vi "Update Stats.vi"(6 "ACK Errors":u32, 8 "error in (no error)":errorcluster, 9 "Number Read":i32, 10 "Number Filtered":u32, 11 "CAN_RW_CORE in":refnum<class "CAN_RW_CORE.lvclass">) -> (0 "error out":errorcluster, 3 "CAN_RW_CORE out":refnum<class "CAN_RW_CORE.lvclass">)   [LabVIEW 2021, in "CAN_RW_CORE.lvclass"]
uses:
  CAN_RW_CORE.lvclass
  CAN_RW_CORE.lvclass/CAN_RW_CORE.ctl
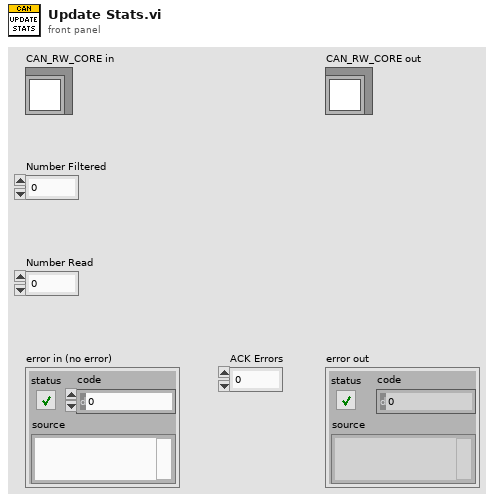
[diagram p1: front panel]
types:
  T1 = typedef "CAN_RW_CORE.lvclass/Statistics.ctl" = cluster{"Total Frames RW":u32, "Frames Filtered ":u32, "ACK Errors":u32}
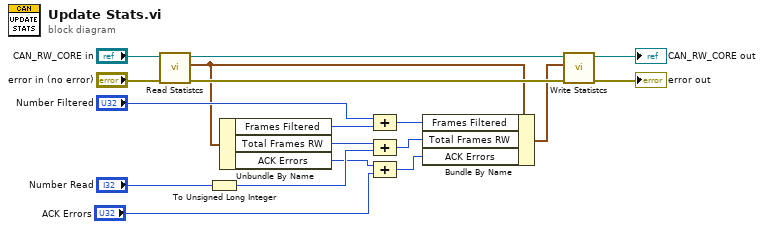
[diagram p0: block diagram]
diagram:
  n1 = call "Read Statistcs.vi"("error in (no error)"="error in (no error)", "CAN_RW_CORE in"="CAN_RW_CORE in") -> ("error out"=w15:errorcluster, "Statistcs"=w10:T1, "CAN_RW_CORE out"=w11:refnum<class "CAN_RW_CORE.lvclass">)  [unwired: 7 in]
  n2 = To Unsigned Long Integer(number="Number Read") -> (unsigned 32bit integer=w7:u32)
  n3 = Unbundle By Name(w10) -> ("Frames Filtered"=w5:u32, "Total Frames RW"=w9:u32, "ACK Errors"=w3:u32)
  n4 = Compound Arithmetic op=ADD("Number Filtered", w5) -> (w4:u32)
  n5 = Compound Arithmetic op=ADD(w9, w7) -> (w8:u32)
  n6 = Compound Arithmetic op=ADD(w3, "ACK Errors") -> (w2:u32)
  n7 = Bundle By Name(cluster=w10, "Frames Filtered"=w4, "Total Frames RW"=w8, "ACK Errors"=w2) -> (w6:T1)
  n8 = call "Write Statistcs.vi"("error in (no error)"=w15, "Statistcs"=w6, "CAN_RW_CORE in"=w11) -> ("error out"=→"error out":errorcluster, "CAN_RW_CORE out"=→"CAN_RW_CORE out":refnum<class "CAN_RW_CORE.lvclass">)  [unwired: 7 in]
